vi "get channels.vi"(11 "module configuration in":refnum<class "TDMS datalogger configuration.lvclass">) -> (2 "channels":refnum<class "TBM channel.lvclass">[](array[class]), 3 "module configuration out":refnum<class "TDMS datalogger configuration.lvclass">)   [LabVIEW 2015, in "TDMS datalogger configuration.lvclass"]
uses:
  TDMS datalogger configuration.lvclass
  <vilib>/NI/Tag Bus Module Framework/channel/TBM channel.lvclass
  TDMS datalogger configuration.lvclass/TDMS datalogger configuration.ctl
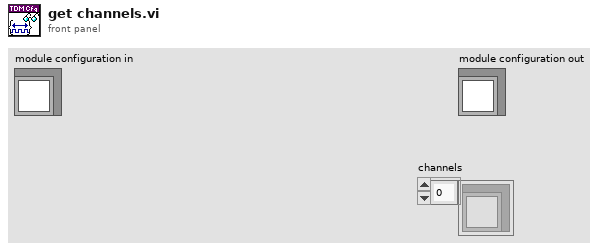
[diagram p1: front panel]
types:
  T1 = cluster{"channel":refnum<class "TBM channel.lvclass">}[]
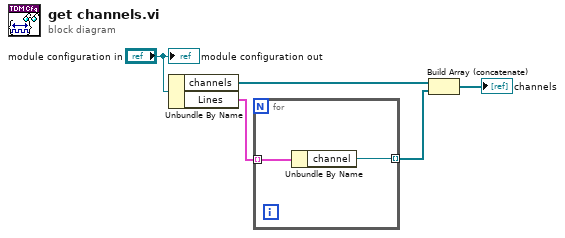
[diagram p0: block diagram]
diagram:
  n1 = Unbundle By Name("module configuration in") -> ("channels"=w4:refnum<class "TBM channel.lvclass">[], "Lines"=w3:T1)
  n2 = for {
    tunnel: w3 -> [w7] mode=indexing
    tunnel: [w6] -> w1 mode=indexing
    n3 = Unbundle By Name(w7) -> ("channel"=w6:refnum<class "TBM channel.lvclass">)
  }
  n4 = Build Array (concatenate)(w4, w1) -> (→"channels":refnum<class "TBM channel.lvclass">[])
  "module configuration out" <- "module configuration in"
